vi "initialize Mast Device.vi"(8 "error in (no error)":errorcluster, 10 "VISA resource name":refnum<visa-resource-name>, 11 "Interface - Mast in":refnum<class "Interface - Mast.lvclass">) -> (0 "error out":errorcluster, 3 "Interface - Mast out":refnum<class "Interface - Mast.lvclass">)   [LabVIEW 2023, in "Turn Table and Mast.lvlib" / "Interface - Mast.lvclass"]
uses:
  Interface - Mast.lvclass
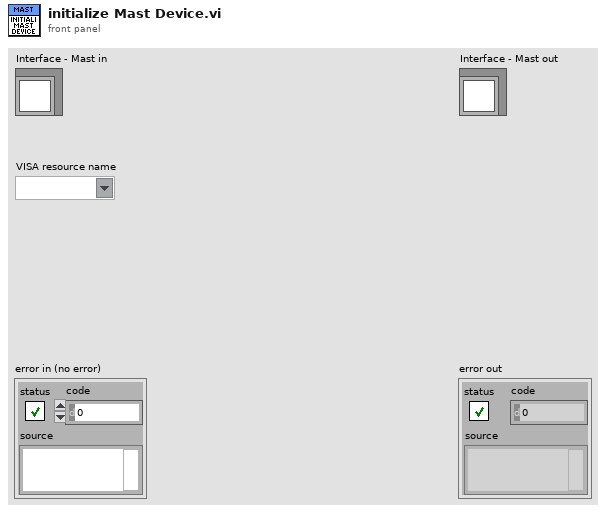
[diagram p1: front panel]
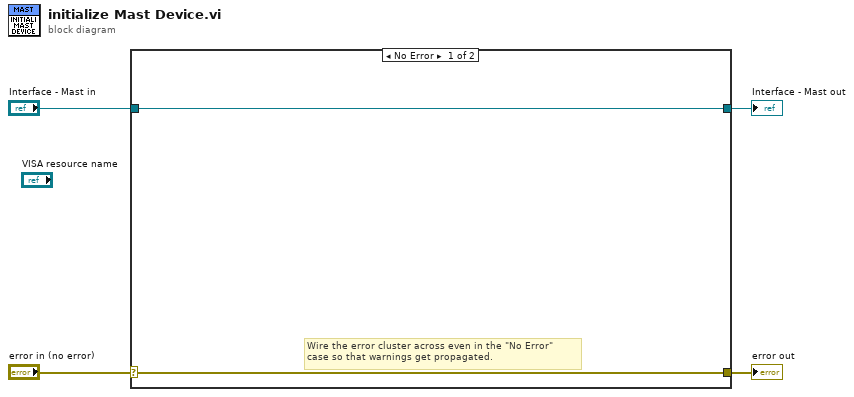
[diagram p0: block diagram]
diagram:
  n1 = case shown="No Error" "error in (no error)" {
    selector: "error in (no error)" -> [w5 w8]
    tunnel: [w5 w8] -> w3
    tunnel: [w6 w7] -> w1
    tunnel: "Interface - Mast in" -> [w6 w7]
    frame No Error {
      # "Wire the error cluster across even in the \"No Error\"\ncase so that warnings get propagated."
    }
    frame Error {
    }
  }
  "error out" <- w3
  "Interface - Mast out" <- w1
